vi "RemoteVI Read Splitters.vi"(0 "VI":refnum<vi>, 1 "refresh?":bool, 2 "origin":cluster{"x":i32, "y":i32}, 3 "message in":string="splitters []", 5 "bars in":T1(array[cluster])) -> (4 "message out":string, 6 "bars out":T1(array[cluster]), 15 "error out":errorcluster)   [LabVIEW 2020, in "RemoteVI.lvlib"]
doc: "Reads the splitter bars of the published panel for the splitters message (docs\\protocol.md 3.3) - LabVIEW moves a splitter bar only while it tracks the real mouse, so the browser drags the bars itself and the server sets the new position (RemoteVI Apply Splitter.vi). When refresh? is TRUE (right after a geometry refresh or a splitter move, never while a popup or a modal window is open, because these are VI Server calls that would block in their modal loop) every bar of {LV.Panel} Splitters[] gives one entry: the area the splitter divides starts at its GObject Position (panel coordinates), the bar lies Splitter Position pixels into it (to the right for a vertical bar, down for a horizontal one) and is GObject Bounds wide and high. Its top-left is converted to screen coordinates (CvtPanelToScreenCoords) and then to frame coordinates (minus the top-left of Front Panel Window:Panel Bounds, plus origin). min is where the area starts in the frame, max where the bar's edge may go at most (the end of the panel area minus the bar's thickness); LabVIEW keeps its own minimum pane sizes when the position is set. bars out keeps the bars for RemoteVI Apply Splitter.vi; RemoteVI Splitters Message.vi builds message out. Otherwise, or on an error, message out and bars out are message in and bars in."
uses:
  RemoteVI.lvlib
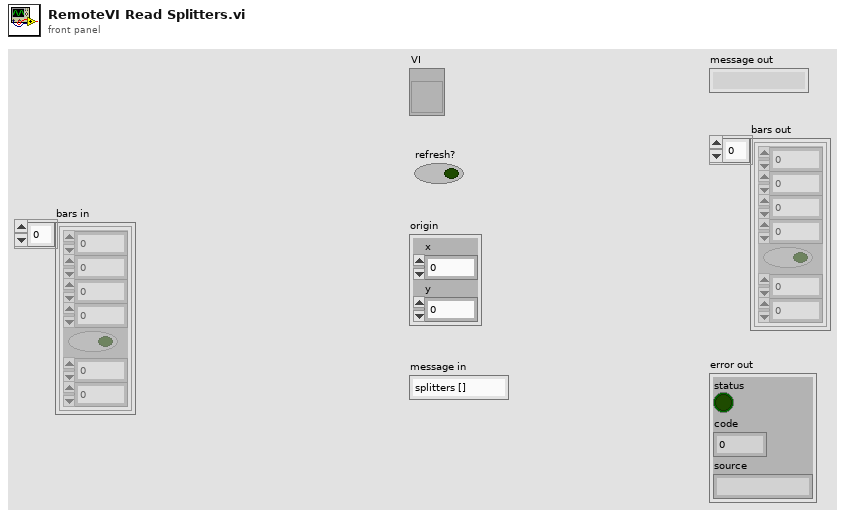
[diagram p1: front panel]
types:
  T1 = cluster{"x":i32, "y":i32, "w":i32, "h":i32, "vertical":bool, "min":i32, "max":i32}[]
  T2 = cluster{"x":i32, "y":i32, "w":i32, "h":i32, "vertical":bool, "min":i32, "max":i32}
  T3 = typedef "LVRectTypeDef.ctl" = cluster{"left":i16, "top":i16, "right":i16, "bottom":i16}
  T4 = typedef "LVPositionTypeDef.ctl" = cluster{"Left":i32, "Top":i32}
  T5 = typedef "LVBoundsTypeDef.ctl" = cluster{"Width":u32, "Height":u32}
  T6 = typedef "LVPointTypeDef.ctl" = cluster{"Horizontal":i16, "Vertical":i16}
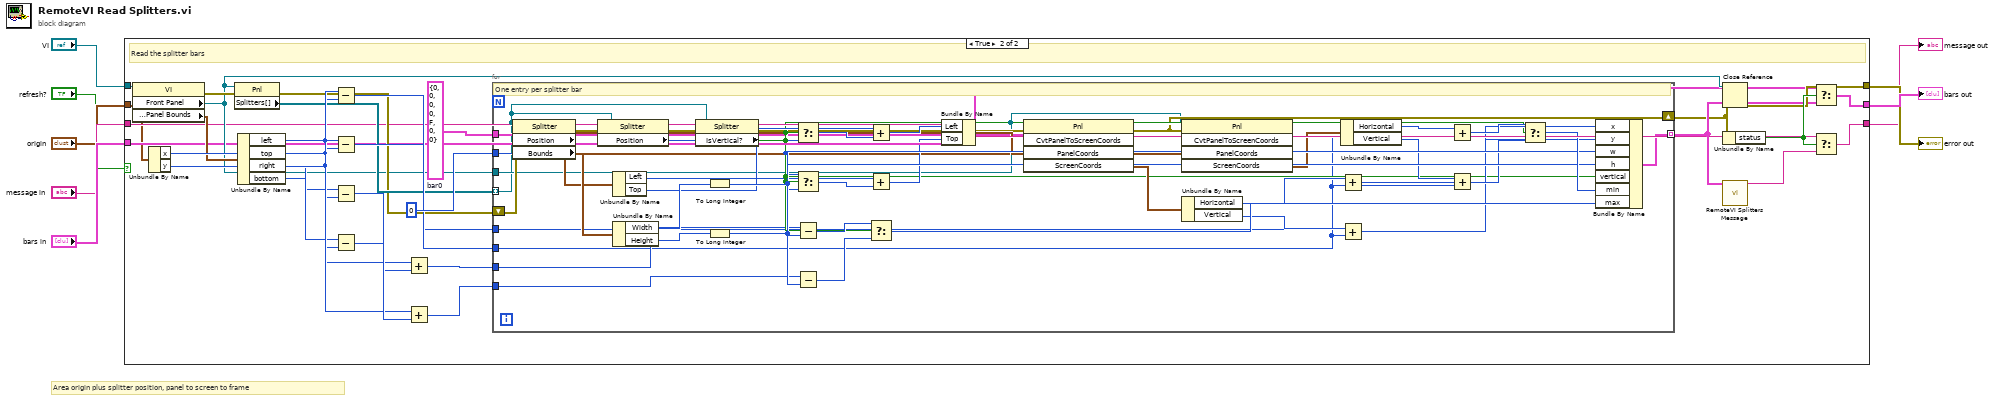
[diagram p0: block diagram]
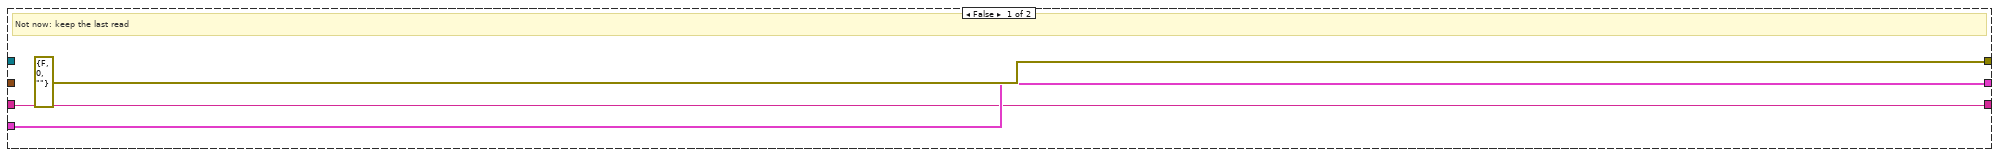
[diagram p2: hidden frame]
diagram:
  # "Area origin plus splitter position, panel to screen to frame"
  n1 = case shown="True" "refresh?" {
    tunnel: "VI" -> [_ w12]
    tunnel: "origin" -> [_ w13]
    tunnel: "message in" -> [w9 w14]
    tunnel: "bars in" -> [w10 w15]
    tunnel: [errorcluster {"status"=FALSE, "code"=0, "source"=""} w37] -> w7
    tunnel: [w10 w41] -> w8
    tunnel: [w9 w40] -> w6
    frame False {
      # "Not now: keep the last read"
    }
    frame True {
      w33 = T2 {"x"=0, "y"=0, "w"=0, "h"=0, "vertical"=FALSE, "min"=0, "max"=0}  # bar0
      # "Read the splitter bars"
      n2 = property class="VI"(reference=w12) -> (error out=w18:errorcluster, "Front Panel"=w16:refnum<vi>, "Front Panel Window:Panel Bounds"=w17:T3)  [unwired: 1 in, 1 out]
      n3 = Unbundle By Name(w13) -> ("x"=w25:i32, "y"=w26:i32)
      n4 = property class="Pnl"(reference=w16, error in=w18) -> (error out=w19:errorcluster, "Splitters[]"=w20:refnum<vi>[])  [unwired: 1 out]
      n5 = Unbundle By Name(w17) -> ("left"=w21:i16, "top"=w22:i16, "right"=w23:i16, "bottom"=w24:i16)
      n6 = Subtract(x=w25, y=w21) -> (x-y=w27:i32)
      n7 = Subtract(x=w26, y=w22) -> (x-y=w28:i32)
      n8 = Subtract(x=w23, y=w21) -> (x-y=w29:i16)
      n9 = Subtract(x=w24, y=w22) -> (x-y=w30:i16)
      n10 = Add(x=w25, y=w29) -> (x+y=w31:i32)
      n11 = Add(x=w26, y=w30) -> (x+y=w32:i32)
      n12 = for {
        tunnel: w33 -> [w45]
        tunnel: 0 -> [w49]
        tunnel: w16 -> [w46]
        tunnel: w20 -> [w42] mode=indexing
        shift-right: [w51] -> w35
        shift-left: w19 -> [w50]
        tunnel: w27 -> [w43]
        tunnel: w28 -> [w44]
        tunnel: w31 -> [w47]
        tunnel: w32 -> [w48]
        tunnel: [w84] -> w36 mode=indexing
        # "One entry per splitter bar"
        n13 = property class="Splitter"(reference=w42, error in=w50) -> (error out=w54:errorcluster, "Position"=w52:T4, "Bounds"=w53:T5)  [unwired: 1 out]
        n14 = property class="Splitter"(reference=w42, error in=w54) -> (error out=w55:errorcluster, "Position"=w56:i32)  [unwired: 1 out]
        n15 = Unbundle By Name(w52) -> ("Left"=w59:i32, "Top"=w60:i32)
        n16 = Unbundle By Name(w53) -> ("Width"=w61:u32, "Height"=w62:u32)
        n17 = property class="Splitter"(reference=w42, error in=w55) -> (error out=w57:errorcluster, "IsVertical?"=w58:bool)  [unwired: 1 out]
        n18 = To Long Integer(number=w61) -> (32bit integer=w78:i32)
        n19 = To Long Integer(number=w62) -> (32bit integer=w79:i32)
        n20 = Select(t=w56, s=w58, f=w49) -> (s? t:f=w63:i32)
        n21 = Select(t=w49, s=w58, f=w56) -> (s? t:f=w64:i32)
        n22 = Subtract(x=w47, y=w78) -> (x-y=w80:i32)
        n23 = Subtract(x=w48, y=w79) -> (x-y=w81:i32)
        n24 = Add(x=w59, y=w63) -> (x+y=w65:i32)
        n25 = Add(x=w60, y=w64) -> (x+y=w66:i32)
        n26 = Select(t=w80, s=w58, f=w81) -> (s? t:f=w83:i32)
        n27 = Bundle By Name(cluster=w52, "Left"=w65, "Top"=w66) -> (w67:T4)
        n28 = invoke class="Pnl" method="CvtPanelToScreenCoords"(reference=w46, error in=w57, "PanelCoords"=w67) -> (error out=w51:errorcluster, "ScreenCoords"=w68:T6)  [unwired: 2 in, 3 out]
        n29 = invoke class="Pnl" method="CvtPanelToScreenCoords"(reference=w46, error in=w51, "PanelCoords"=w52) -> ("ScreenCoords"=w69:T6)  [unwired: 2 in, 4 out]
        n30 = Unbundle By Name(w68) -> ("Horizontal"=w70:i16, "Vertical"=w71:i16)
        n31 = Unbundle By Name(w69) -> ("Horizontal"=w72:i16, "Vertical"=w73:i16)
        n32 = Add(x=w70, y=w43) -> (x+y=w74:i32)
        n33 = Add(x=w71, y=w44) -> (x+y=w75:i32)
        n34 = Add(x=w72, y=w43) -> (x+y=w76:i32)
        n35 = Add(x=w73, y=w44) -> (x+y=w77:i32)
        n36 = Select(t=w76, s=w58, f=w77) -> (s? t:f=w82:i32)
        n37 = Bundle By Name(cluster=w45, "x"=w74, "y"=w75, "w"=w78, "h"=w79, "vertical"=w58, "min"=w82, "max"=w83) -> (w84:T2)
      }
      n38 = Close Reference(reference=w16, error in (no error)=w35) -> (error out=w37:errorcluster)
      n39 = Unbundle By Name(w35) -> ("status"=w39:bool)
      n40 = call "RemoteVI Splitters Message.vi"("bars"=w36) -> ("message"=w38:string)  [unwired: 14 in]
      n41 = Select(t=w15, s=w39, f=w36) -> (s? t:f=w41:T1)
      n42 = Select(t=w14, s=w39, f=w38) -> (s? t:f=w40:string)
    }
  }
  "message out" <- w6
  "bars out" <- w8
  "error out" <- w7
